vi "_Raise Source Changed Event.vi"(4 "WebView2.lvlib:WebView2 Control.lvclass":refnum<class "WebView2 Control.lvclass">, 5 "Event Data":cluster{"sender":refnum<k24>, "e":refnum<k24>}, 6 "Control Ref":refnum<k24>, 7 "Event Common Data":T1) -> ()   [LabVIEW 2020, in "WebView2.lvlib" / "WebView2 Control.lvclass"]
uses:
  WebView2 Control.lvclass
  E:/Labview/LV 2023/PPL/PPL Builder/Libs/LV-WebView2/Source/Libs/Microsoft.Web.WebView2.Core.dll
  Libs/Microsoft.Web.WebView2.Core.dll
  WebView2 Control.lvclass/WebView2 Control.ctl
  WebView2 Event Filter Interface/WebView2 Event Filter Interface.lvclass
  Source Changed Event Data.ctl
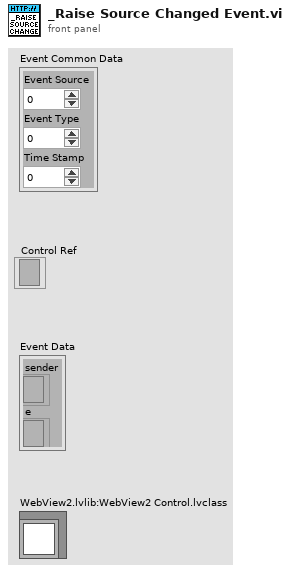
[diagram p1: front panel]
types:
  T1 = cluster{"Event Source":i32, "Event Type":u32, "Time Stamp":u32}
  T2 = typedef "WebView2.lvlib/WebView2 Control.lvclass/Source Changed Event Data.ctl" = cluster{"Source":string, "IsNewDocument":bool}
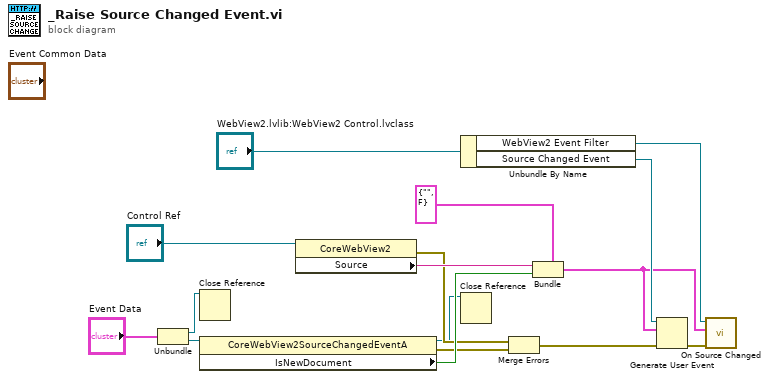
[diagram p0: block diagram]
diagram:
  n1 = Unbundle("Event Data") -> ("sender"=w5:refnum<k24>, "e"=w13:refnum<k24>)
  n2 = Close Reference(reference=w5) -> ()  [unwired: 1 in, 1 out]
  n3 = property class="CoreWebView2SourceChangedEventA"(reference=w13) -> (reference out=w4:refnum<k24>, error out=w8:errorcluster, "IsNewDocument"=w11:bool)  [unwired: 1 in]
  n4 = property class="CoreWebView2"(reference="Control Ref") -> (error out=w6:errorcluster, "Source"=w9:string)  [unwired: 1 in, 1 out]
  n5 = Unbundle By Name("WebView2.lvlib:WebView2 Control.lvclass") -> ("WebView2 Event Filter"=w3:refnum<class "WebView2 Event Filter Interface.lvclass">, "Source Changed Event"=w15:refnum<user-event>)
  n6 = Close Reference(reference=w4) -> ()  [unwired: 1 in, 1 out]
  n7 = Merge Errors(w6, w8) -> (w7:errorcluster)
  n8 = Bundle(cluster=T2 {"Source"="", "IsNewDocument"=FALSE} ("output cluster"), "Source"=w9, "IsNewDocument"=w11) -> (w2:T2)
  n9 = Generate User Event(user event=w15, event data cluster=w2, error in=w7) -> (error out=w1:errorcluster)  [unwired: 1 in, 1 out]
  n10 = call-dynamic "On Source Changed.vi"("error in (no error)"=w1, "Data"=w2, "WebView2 Event Filter Interface in"=w3) -> ()  [unwired: 8 in, 1 out]
